vi "nominal close.vi"(11 "connection":refnum<class "Nominal Client.lvclass">) -> (0 "error out":errorcluster)   [LabVIEW 2020, in "nominal core steps.lvlib"]
doc: "Closes the connection to Nominal\n<b> </b> <b> </b>"
uses:
  nominal core steps.lvlib
  <vilib>/Nominal/Nominal IO Client/lv_src/Nominal Client/Nominal Client.lvclass
  <vilib>/Nominal/Nominal IO Client/lv_src/Nominal Client/Nominal Client.lvclass/Nominal Client.ctl
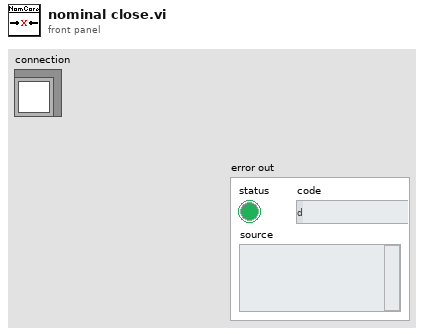
[diagram p1: front panel]
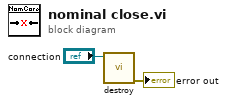
[diagram p0: block diagram]
diagram:
  n1 = call <vilib>:"destroy.vi"("Nominal Client"="connection") -> ("error out"=→"error out":errorcluster)  [unwired: 10 in]
